vi "sinlge_motor.vi"() -> ()   [LabVIEW 2023]
uses:
  <instrlib>/Phidgets/Phidget Voltage Ratio Input/Public/VoltageRatioInputStart.vi
  <instrlib>/Phidgets/Phidget Voltage Ratio Input/Public/VoltageRatioInputClose.vi
  <instrlib>/Phidgets/Phidget Common/Phidget Common.lvlib
  <instrlib>/Phidgets/Phidget Voltage Ratio Input/Phidget Voltage Ratio Input.lvlib
panel:
  in  "stop":bool
  in  "Max Torque":dbl
  in  "Velocity":dbl
  in  "IsHubPort":bool
  out "Serial Number Return":i32
  in  "Device Info":T1={"Serial Number"=-1, "Channel"=0, "Port"=0}
  out "error out":errorcluster
  out "Voltage Ratio":dbl format="%_4g"
  out "Torque":dbl
  in  "Torque":dbl
  in  "Position":dbl
  out "main error":errorcluster
  out "Position":dbl
  in  "Control Selection":T2(ring)
  out "Close session error":errorcluster
  out "start error":errorcluster
  out "iter":dbl
  in  "?":bool
  # "Motor Telemetry"
  # "Motor Controls"
  # "Move Controls"
  # "Load Cell Output"
  # "Velocity Torque Max Controls"
  # "Torque Control"
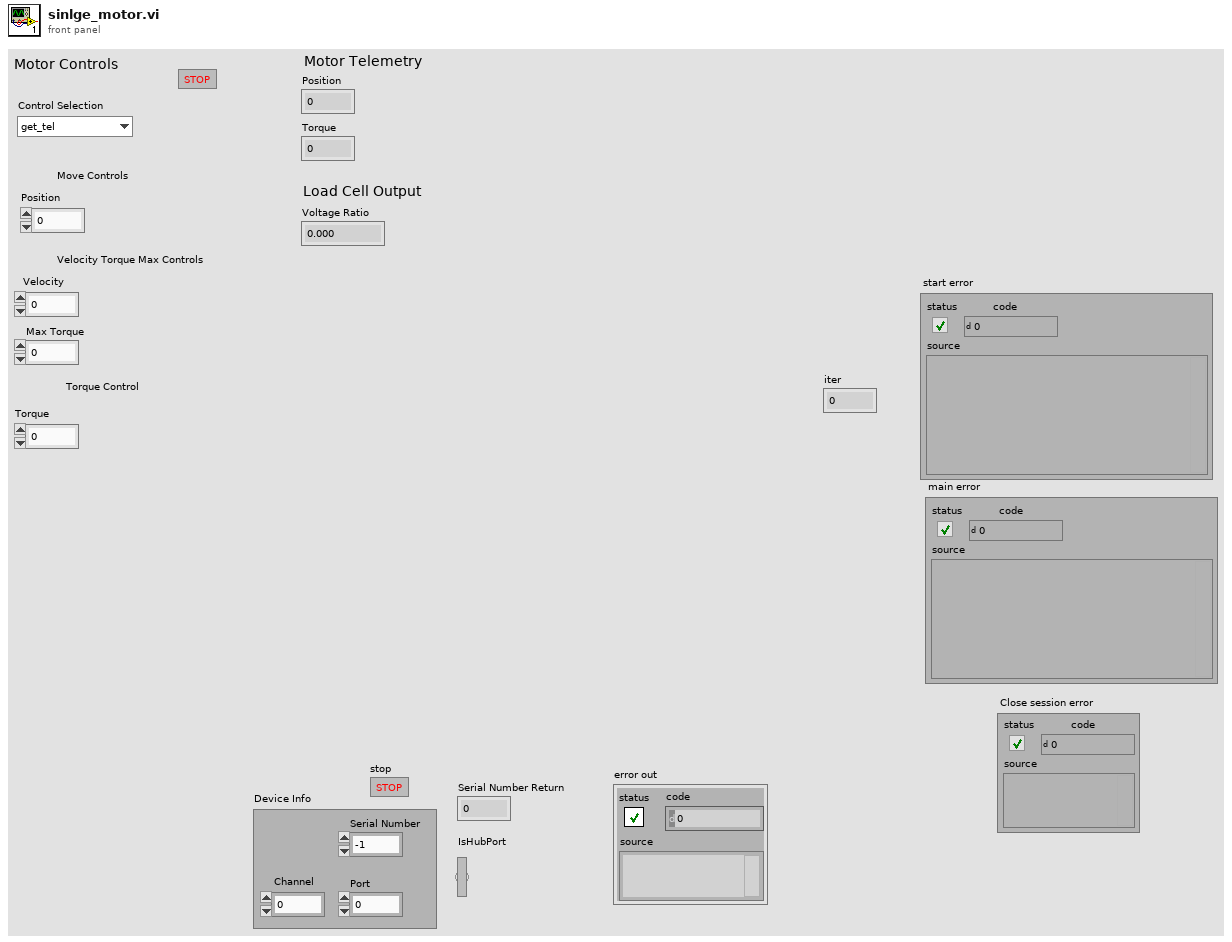
[diagram p1: front panel]
types:
  T1 = cluster{"Serial Number":i32, "Channel":i32, "Port":i32}
  T2 = enum16{"get_tel", "hold", "move", "vel_trq", "torque"}
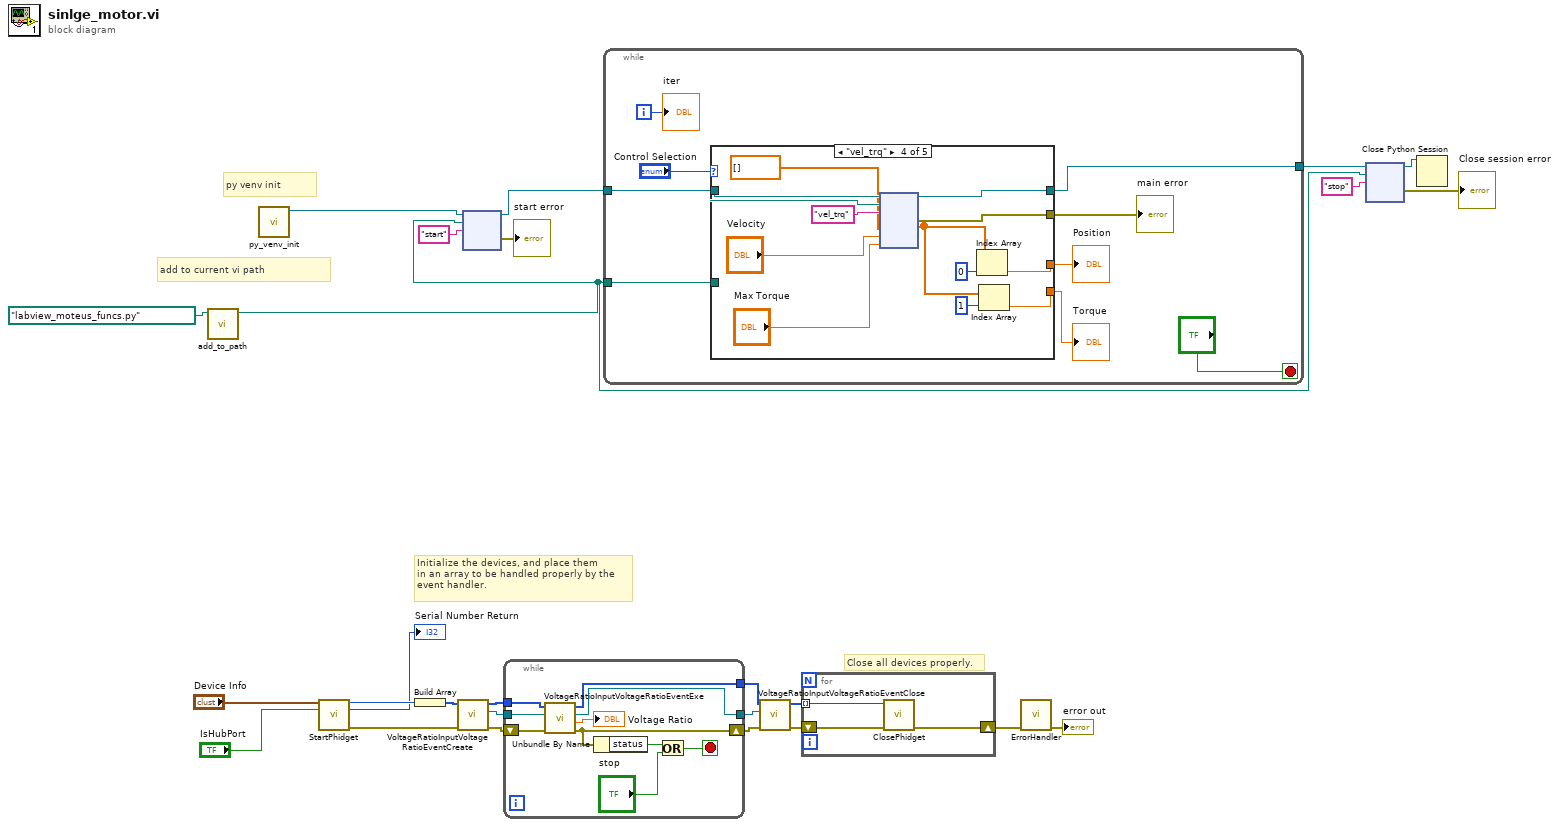
[diagram p0: block diagram]
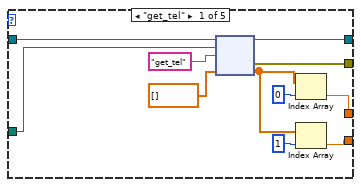
[diagram p2: hidden frame]
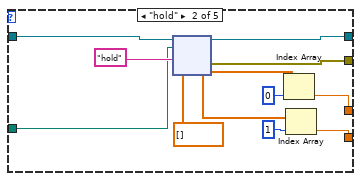
[diagram p3: hidden frame]
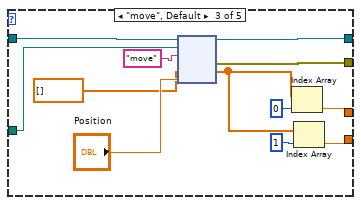
[diagram p4: hidden frame]
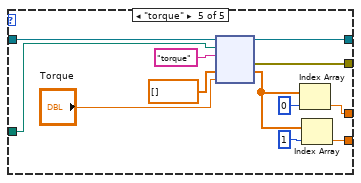
[diagram p5: hidden frame]
diagram:
  # "add to current vi path"
  # "py venv init"
  # "Close all devices properly."
  # "Initialize the devices, and place them\nin an array to be handled properly by the\nevent handler."
  n1 = call "add_to_path.vi"("Path"=path "labview_moteus_funcs.py") -> ("appended path"=w1:path)  [unwired: 10 in]
  n2 = call "py_venv_init.vi"() -> ("Refnum out"=w24:refnum<k35>)  [unwired: 11 in]
  n3 = call-poly <instrlib>:"StartPhidget.vi"("Device Info"="Device Info", "IsHubPort"="IsHubPort") -> ("Phidget ID"=w8:u64, "Serial Number Return"=→"Serial Number Return":i32, "error out"=w4:errorcluster)  [unwired: 10 in, 1 out]
  n4 = Build Array(w8) -> (w18:u64[])
  n5 = call <instrlib>:"VoltageRatioInputVoltageRatioEventCreate.vi"("error in (no error)"=w4, "Devices In"=w18) -> ("error out"=w11:errorcluster, "Event Registration Refnum"=w16:refnum<event-registration>, "Devices Out"=w17:u64[])  [unwired: 7 in]
  n6 = node(w24, w1, "start") -> (w23:refnum<k35>, →"start error":errorcluster)  [unwired: 3 in, 2 out]
  n7 = while {
    tunnel: w17 -> [w36]
    tunnel: w16 -> [w32]
    tunnel: [w35] -> w13
    shift-right: [w31] -> w12
    shift-left: w11 -> [w34]
    tunnel: [w33] -> w6
    stop <- w30 stop-if-true
    n8 = call <instrlib>:"VoltageRatioInputVoltageRatioEventExe.vi"("error in (no error)"=w34, "Event Registration Refnum In"=w32, "Devices In"=w36) -> ("error out"=w31:errorcluster, "VoltageRatio"=→"Voltage Ratio":dbl, "Event Registration Refnum Out"=w35:refnum<event-registration>, "Devices Out"=w33:u64[])  [unwired: 2 in, 3 out]
    n9 = Unbundle By Name(w31) -> ("status"=w29:bool)
    n10 = Or(x=w29, y="stop") -> (x .or. y?=w30:bool)
  }
  n11 = while {
    tunnel: [w44] -> w22
    tunnel: w23 -> [w43]
    tunnel: w1 -> [w42]
    i -> [w45]
    stop <- "?" stop-if-true
    n12 = case shown="\"vel_trq\"" "Control Selection" {
      tunnel: [w56 w67 w79 w92 w104] -> w44
      tunnel: w43 -> [w54 w65 w77 w90 w102]
      tunnel: [w53 w64 w75 w88 w101] -> w40
      tunnel: w42 -> [w52 w63 w74 w87 w100]
      tunnel: [w47 w57 w68 w81 w95] -> w38
      tunnel: [w46 w58 w69 w80 w94] -> w37
      frame "get_tel" {
        n13 = node(w54, w52, "get_tel", dbl[] []) -> (w56:refnum<k35>, w53:errorcluster, w48:dbl[])  [unwired: 1 in, 2 out]
        n14 = Index Array(array=w48, index=0) -> (element=w46:dbl)
        n15 = Index Array(array=w48, index=1) -> (element=w47:dbl)
      }
      frame "hold" {
        n16 = node(w65, w63, "hold", dbl[] []) -> (w67:refnum<k35>, w64:errorcluster, w59:dbl[])  [unwired: 1 in, 2 out]
        n17 = Index Array(array=w59, index=0) -> (element=w58:dbl)
        n18 = Index Array(array=w59, index=1) -> (element=w57:dbl)
      }
      frame "move", Default {
        n19 = node(w77, w74, "move", dbl[] [], "Position") -> (w79:refnum<k35>, w75:errorcluster, w70:dbl[])  [unwired: 2 in, 2 out]
        n20 = Index Array(array=w70, index=0) -> (element=w69:dbl)
        n21 = Index Array(array=w70, index=1) -> (element=w68:dbl)
      }
      frame "vel_trq" {
        n22 = node(w90, w87, "vel_trq", dbl[] [], "Velocity", "Max Torque") -> (w92:refnum<k35>, w88:errorcluster, w82:dbl[])  [unwired: 3 in, 2 out]
        n23 = Index Array(array=w82, index=0) -> (element=w80:dbl)
        n24 = Index Array(array=w82, index=1) -> (element=w81:dbl)
      }
      frame "torque" {
        n25 = node(w102, w100, "torque", dbl[] [], "Torque") -> (w104:refnum<k35>, w101:errorcluster, w96:dbl[])  [unwired: 2 in, 2 out]
        n26 = Index Array(array=w96, index=0) -> (element=w94:dbl)
        n27 = Index Array(array=w96, index=1) -> (element=w95:dbl)
      }
    }
    "main error" <- w40
    "Torque" <- w38
    "Position" <- w37
    "iter" <- w45
  }
  n28 = call <instrlib>:"VoltageRatioInputVoltageRatioEventClose.vi"("error in (no error)"=w12, "Event Registration Refnum In"=w13, "Devices In"=w6) -> ("error out"=w9:errorcluster, "Devices Out"=w7:u64[])  [unwired: 7 in]
  n29 = for {
    tunnel: w7 -> [w105] mode=indexing
    shift-right: [w107] -> w15
    shift-left: w9 -> [w106]
    n30 = call-poly <instrlib>:"ClosePhidget.vi"("error in"=w106, "Device In"=w105) -> ("error out"=w107:errorcluster)  [unwired: 9 in]
  }
  n31 = call <instrlib>:"ErrorHandler.vi"("error in"=w15) -> ("error out"=→"error out":errorcluster)  [unwired: 9 in, 1 out]
  n32 = node(w22, w1, "stop") -> (w21:refnum<k35>, →"Close session error":errorcluster)  [unwired: 3 in, 2 out]
  n33 = Close Python Session(session in=w21) -> ()  [unwired: 1 in, 1 out]
